vi "CSV_REPORT.vi"(0 "Voltage":string="0", 1 "LO SET":string="0", 2 "HI SET":string="0", 3 "MESURED":string="0", 4 "MEASURED Voltage":string="0", 5 "Result":bool=TRUE, 8 "Result":string[][](array[string])) -> ()   [LabVIEW 2021]
uses:
  Control/Reporting.ctl
  <vilib>/Utility/file.llb/Write Delimited Spreadsheet (string).vi
  <vilib>/Utility/file.llb/Write Delimited Spreadsheet (DBL).vi
panel:
  out "output array 3":string[][](array[string])
  out "output array 2":string[][](array[string])
  out "output array":string[][](array[string])
  out "new file path (Not A Path if cancelled) 2":path
  out "new path 2":path
  out "new path":path
  out "stripped path":path
  out "appended path":path
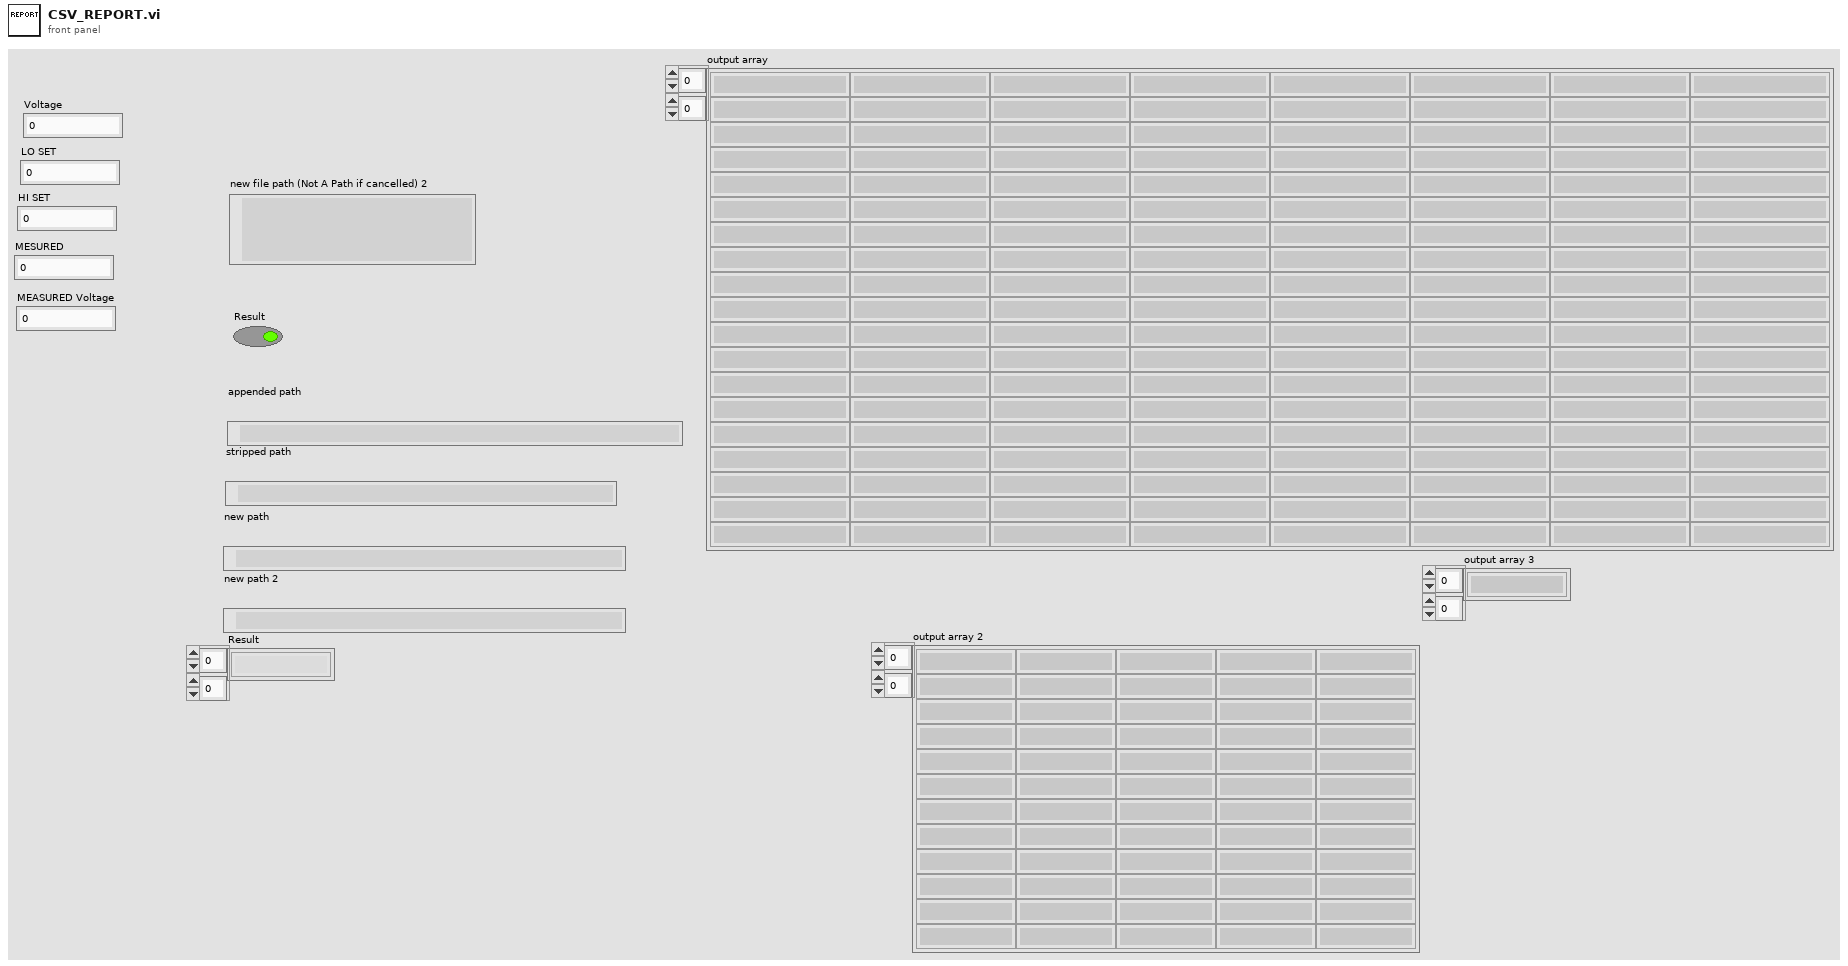
[diagram p1: front panel]
types:
  T1 = typedef "Reporting.ctl" = enum16{"Report Name & Path", "Write Details in report", "Write Test Details in report", "Exit"}
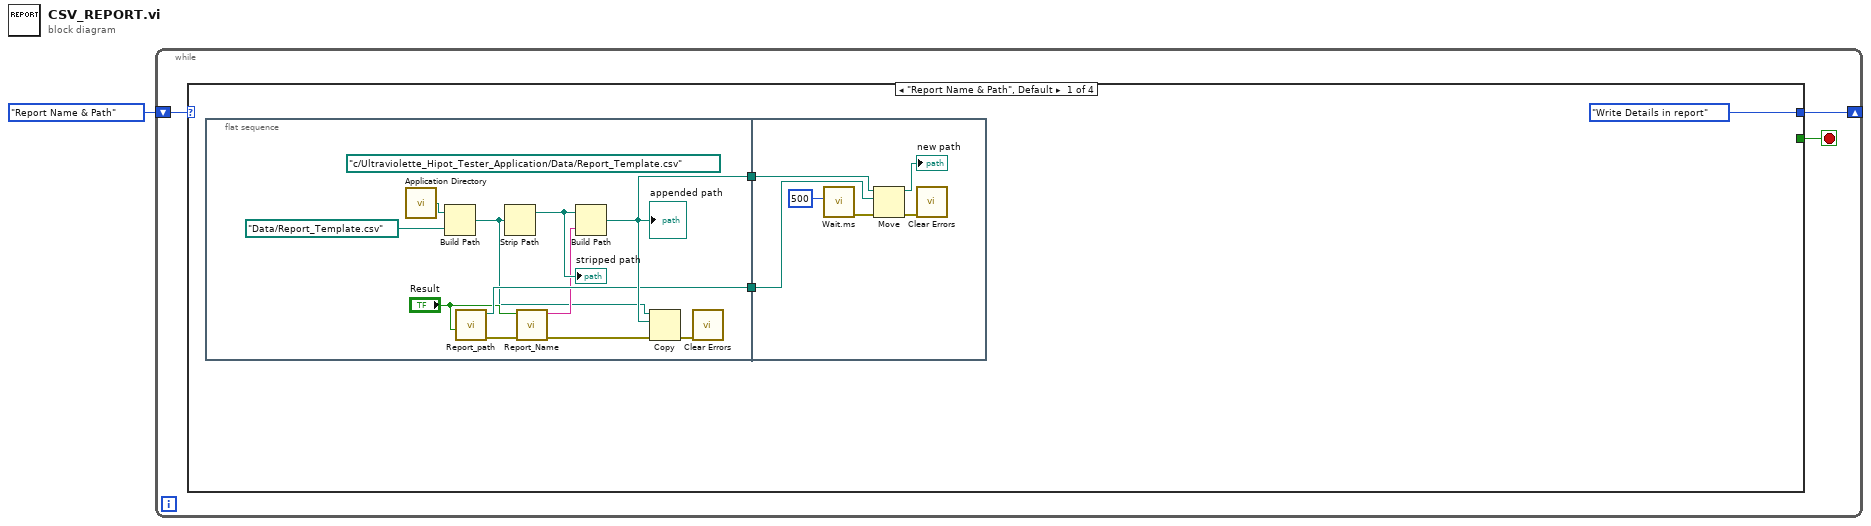
[diagram p0: block diagram]
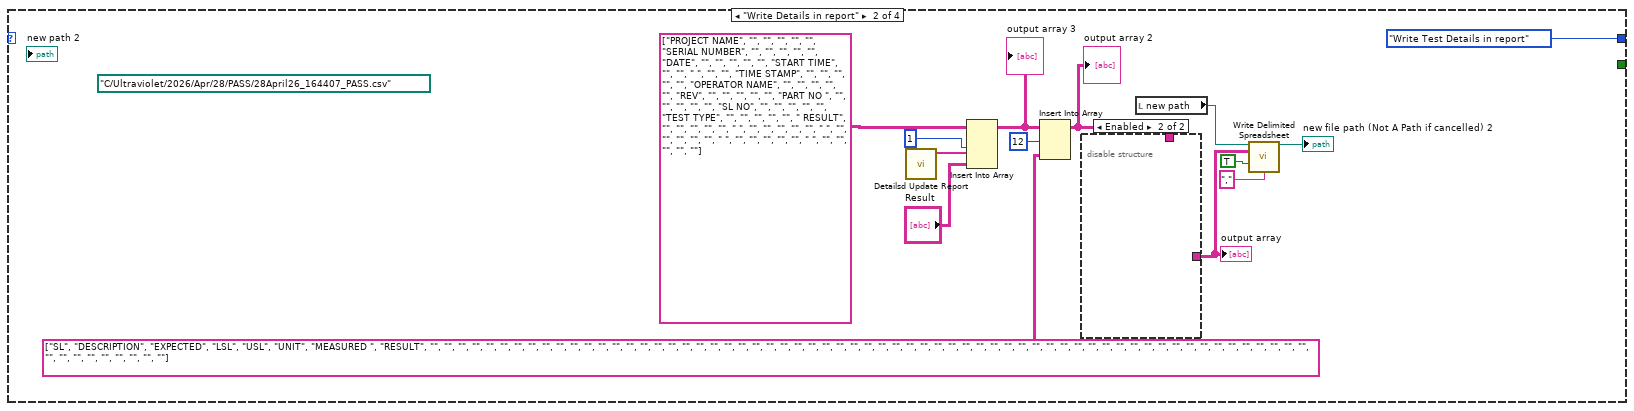
[diagram p2: hidden frame]
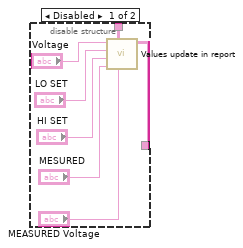
[diagram p3: hidden frame]
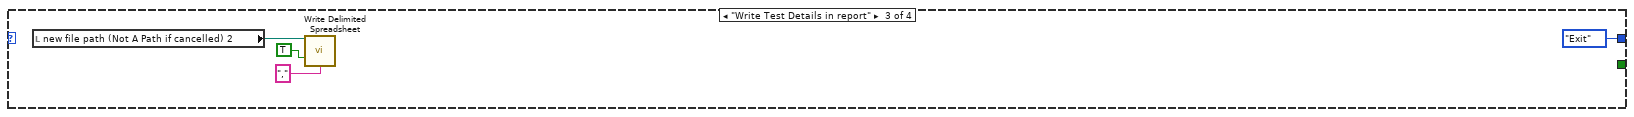
[diagram p4: hidden frame]
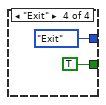
[diagram p5: hidden frame]
diagram:
  n1 = while {
    shift-right: [w3] -> _
    shift-left: Reporting."Report Name & Path" -> [w4]
    stop <- w2 stop-if-true
    n2 = case shown="\"Report Name & Path\", Default" w4 {
      tunnel: [Reporting."Write Details in report" Reporting."Write Test Details in report" Reporting."Exit" Reporting."Exit"] -> w3
      tunnel: [_ _ _ TRUE] -> w2
      frame "Report Name & Path", Default {
        n3 = flat-sequence {
          tunnel: [w16] -> w7
          tunnel: [w15] -> w6
          tunnel: w7 -> [w23]
          tunnel: w6 -> [w22]
          frame #0 {
            (unwired) path "c:/Ultraviolette_Hipot_Tester_Application/Data/Report_Template.csv" ("source path")
            n4 = call <vilib>:"Application Directory.vi"() -> ("Application Directory"=w10:path)
            n5 = Build Path(base path=w10, name or relative path=path "Data/Report_Template.csv") -> (appended path=w8:path)
            n6 = call "Report_path.vi"("Result"="Result") -> ("error out"=w14:errorcluster, "appended path"=w15:path)  [unwired: 9 in]
            n7 = Strip Path(path=w8) -> (stripped path=w18:path)  [unwired: 1 out]
            "stripped path" <- w18
            n8 = call "Report_Name.vi"("error In"=w14, "Result"="Result") -> ("error In"=w12:errorcluster, "Report Name"=w11:string)  [unwired: 8 in]
            n9 = Build Path(base path=w18, name or relative path=w11) -> (appended path=w16:path)
            "appended path" <- w16
            n10 = Copy(8:w12, 10:w16, 11:w8) -> (0:w17:errorcluster)  [unwired: 2 in, 2 out]
            n11 = call <vilib>:"Clear Errors.vi"("error in (no error)"=w17) -> ()  [unwired: 5 in, 2 out]
          }
          frame #1 {
            n12 = call "Wait.ms.vi"("milliseconds to wait"=u32 500) -> ("error out"=w21:errorcluster)  [unwired: 10 in]
            n13 = Move(source path=w23, error in=w21, 10:w22) -> (error out=w24:errorcluster, 3:→"new path":path)  [unwired: 2 in, 1 out]
            n14 = call <vilib>:"Clear Errors.vi"("error in (no error)"=w24) -> ()  [unwired: 5 in, 2 out]
          }
        }
      }
      frame "Write Details in report" {
        (unwired) path "C:/Ultraviolet/2026/Apr/28/PASS/28April26_164407_PASS.csv" ("new path")
        n15 = call "Detailsd Update Report.vi"() -> ("appended array"=w34:string[])  [unwired: 11 in]
        n16 = Insert Into Array(array=string[][] [["PROJECT NAME", "", "", "", "", ""], ["SERIAL NUMBER", "", "", "", "", ""], ["DATE", "", "", "", "", ""], ["START TIME", "", "", " ", "", ""], ["TIME STAMP", "", "", "", "", ""], ["OPERATOR NAME", "", "", "", "", ""], ["REV", "", "", "", "", ""], ["PART NO ", "", "", "", "", ""], ["SL NO", "", "", "", "", ""], ["TEST TYPE", "", "", "", "", ""], [" RESULT", "", "", "", "", ""], [" ", "", "", "", "", ""], [" ", "", "", "", "", ""], [" ", "", "", "", "", ""], [" ", "", "", "", "", ""]], index (col)=1 ("disabled index (col)"), new element #1=w34, new element #2="Result") -> (w30:string[][])  [unwired: 1 in]
        "output array 3" <- w30
        n17 = Insert Into Array(array=w30, index (row)=12, new element=string[][] [["SL", "DESCRIPTION", "EXPECTED", "LSL", "USL", "UNIT", "MEASURED ", "RESULT"], ["", "", "", "", "", "", "", ""], ["", "", "", "", "", "", "", ""], ["", "", "", "", "", "", "", ""], ["", "", "", "", "", "", "", ""], ["", "", "", "", "", "", "", ""], ["", "", "", "", "", "", "", ""], ["", "", "", "", "", "", "", ""], ["", "", "", "", "", "", "", ""], ["", "", "", "", "", "", "", ""]]) -> (w27:string[][])  [unwired: 1 in]
        "output array 2" <- w27
        n18 = disable-structure shown="Enabled" {
          disable-tunnel: w27 -> [w45 _]
          disable-tunnel: [w44 _] -> w26
          frame Disabled {
            n19 = call "Values update in report.vi"("MESURED  Voltage"="MEASURED Voltage", "array"=w45, "MESURED"="MESURED", "HI SET"="HI SET", "LO SET"="LO SET", "Voltage"="Voltage") -> ("output array"=w44:string[][])  [unwired: 5 in]
          }
          frame Enabled {
          }
        }
        "output array" <- w26
        n20 = local read "new path"() -> (w31:path)
        n21 = call-poly <vilib>:"Write Delimited Spreadsheet.vi"("file path (dialog if empty)"=w31, "2D data"=w26, "append to file? (new file:F)"=TRUE, "delimiter (\\t)"="," ("delimiter (\\t)")) -> ("new file path (Not A Path if cancelled)"=→"new file path (Not A Path if cancelled) 2":path)  [unwired: 10 in, 1 out]
      }
      frame "Write Test Details in report" {
        n22 = local read "new file path (Not A Path if cancelled) 2"() -> (w46:path)
        n23 = call-poly <vilib>:"Write Delimited Spreadsheet.vi"("file path (dialog if empty)"=w46, "append to file? (new file:F)"=TRUE, "delimiter (\\t)"="," ("delimiter (\\t)")) -> ()  [unwired: 11 in, 2 out]
      }
      frame "Exit" {
      }
    }
  }
